vi "SA delete DisplayLine.vi"(8 "error in (no error)":errorcluster caption="에러 입력(에러 없음)", 11 "Instrument Manager 입력":refnum<class "Instrument Manager.lvclass">) -> (0 "error out":errorcluster caption="에러 출력", 3 "Instrument Manager 출력":refnum<class "Instrument Manager.lvclass">)   [LabVIEW 2023, in "Instrument Manager.lvclass"]
uses:
  Instrument Manager.lvclass
  Instrument Manager.lvclass/Instrument Manager.ctl
  Module/Spectrum Analyzer/Class/FSV-40N/FSV-40N.lvclass
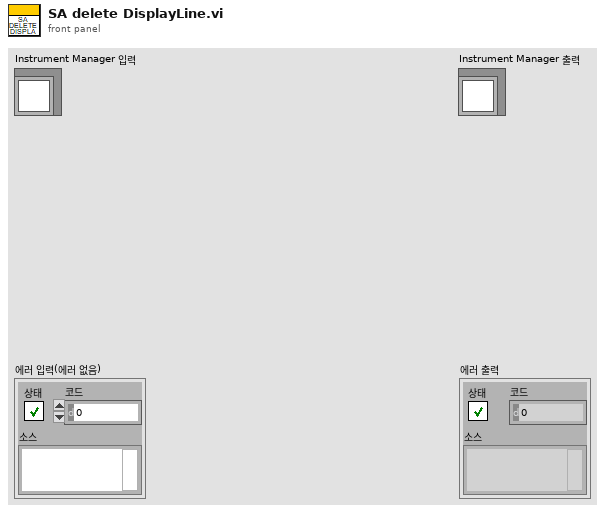
[diagram p1: front panel]
types:
  T1 = cluster{"Anritsu Call Box":refnum<class "Anritsu Call Box.lvclass">, "Spectrum Analyzer":refnum<class "Interface_Spectrum.lvclass">, "RF Switch Box":refnum<class "RF Filter Box.lvclass">, "Turn Table":refnum<class "Interface - Turn Table.lvclass">, "Mast":refnum<class "Interface - Mast.lvclass">, "3D Controller":refnum<class "Interface_3D Controller.lvclass">}
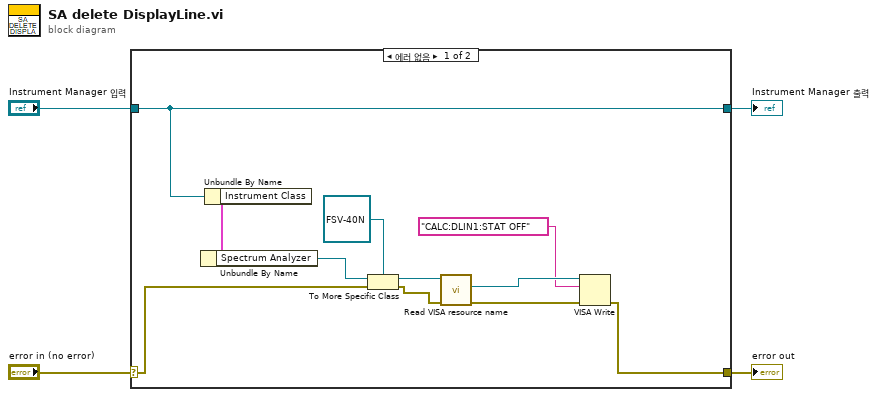
[diagram p0: block diagram]
diagram:
  n1 = case shown="에러 없음" "error in (no error)" {
    selector: "error in (no error)" -> [w12 w17]
    tunnel: [w5 w17] -> w3
    tunnel: [w14 w16] -> w1
    tunnel: "Instrument Manager 입력" -> [w14 w16]
    frame No Error {
      n2 = Unbundle By Name(w14) -> ("Instrument Class"=w15:T1)
      n3 = Unbundle By Name(w15) -> ("Spectrum Analyzer"=w13:refnum<class "Interface_Spectrum.lvclass">)
      n4 = To More Specific Class(target class=refnum<class "FSV-40N.lvclass"> refnum ("Spectrum Analyzer.lvlib:FSV-40N.lvclass"), reference=w13, error in=w12) -> (specific class reference=w10:refnum<class "FSV-40N.lvclass">, error out=w9:errorcluster)
      n5 = call "Read VISA resource name.vi"("error in (no error)"=w9, "FSV-40N in"=w10) -> ("error out"=w8:errorcluster, "VISA resource name"=w7:refnum<visa-resource-name>)  [unwired: 7 in, 1 out]
      n6 = VISA Write(VISA resource name=w7, write buffer="CALC:DLIN1:STAT OFF" ("initial string"), error in (no error)=w8) -> (error out=w5:errorcluster)  [unwired: 2 out]
    }
    frame Error {
    }
  }
  "error out" <- w3
  "Instrument Manager 출력" <- w1
